vi "Send_Msg.vi"(8 "error in (no error)":errorcluster, 9 "NewVal":T1, 10 "action":T2, 11 "Queue in":refnum<queue>) -> (0 "error out":errorcluster, 3 "Queue out":refnum<queue>)   [LabVIEW 2025]
uses:
  vi/thresholds.ctl
  vi/action.ctl
  vi/UI_Msg.ctl
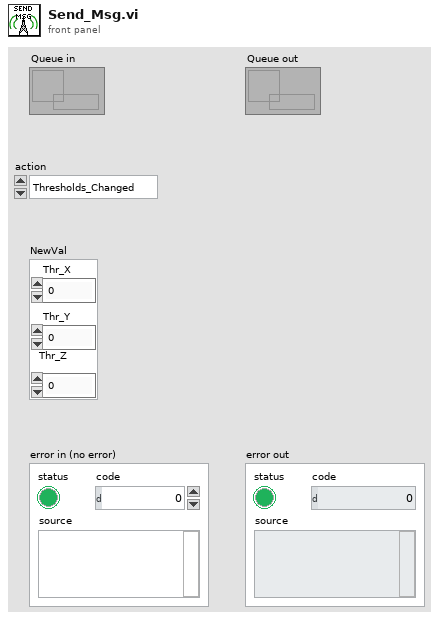
[diagram p1: front panel]
types:
  T1 = typedef "thresholds.ctl" = cluster{"Thr_X":i16, "Thr_Y":i16, "Thr_Z":i16}
  T2 = typedef "action.ctl" = enum16{"Thresholds_Changed", "Manual_Trigger", "Stop"}
  T3 = typedef "UI_Msg.ctl" = cluster{"action":T2, "Threshold":T1}
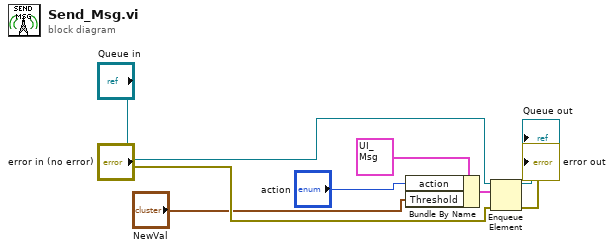
[diagram p0: block diagram]
diagram:
  n1 = Bundle By Name(cluster=T3 {"action"=enum."Thresholds_Changed", "Threshold"={"Thr_X"=0, "Thr_Y"=0, "Thr_Z"=0}} ("msg"), "action"="action", "Threshold"="NewVal") -> (w1:T3)
  n2 = Enqueue Element(queue="Queue in", element=w1, error in (no error)="error in (no error)") -> (queue out=→"Queue out":refnum<queue>, error out=→"error out":errorcluster)  [unwired: 1 in, 1 out]
